vi "TC01 Thermocouple Read.vi"(0 "Physical Channel":tag="Thermocouple1/ai0", 1 "Max Value (deg C)":dbl=100.0, 2 "Min Value (deg C)":dbl, 3 "CJC Source":i32(ring)=10200 items=["Built-In"=10200, "Constant Value"=10116, "Channel"=10113], 4 "CJC Value":dbl=25.0 format="%0.2f", 5 "CJC Channel":refnum<k21>, 6 "Thermocouple Type":i32(ring)=10072 items=["J"=10072, "K"=10073, "N"=10077, "R"=10082, "S"=10085, "T"=10086, "B"=10047, "E"=10055], 7 "Units":i32(ring)=10143 items=["Deg C"=10143, "Deg F"=10144, "Kelvins"=10325, "Deg R"=10145, "From Custom Scale"=10065], 8 "Samples to Average":i32=5 min=1 step=1) -> (20 "Average Read Value":dbl, 21 "Max Read Value":dbl, 22 "Min Read Value":dbl, 23 "Number of reads":i32, 27 "error out":errorcluster)   [LabVIEW 2013]
doc: "This example demonstrates how to continuously acquire temperature measurements using a DAQmx device.\n\nFor instructions on how to connect your signals to the DAQ device, refer to your device documentation."
uses:
  <vilib>/DAQmx/read.llb/DAQmx Read (Analog DBL 1Chan 1Samp).vi
  <vilib>/DAQmx/create/channels.llb/DAQmx Create Channel (AI-Temperature-Thermocouple).vi
  <vilib>/DAQmx/miscellaneous.llb/DAQmx Fill In Error Info.vi
panel:
  out "Approximate\nAcquisition Time":dbl
  out "Waveform Graph":dbl[](graph)
  # "Inputs"
  # "Acquired Data"
  # "Outputs"
  # "Fixed 250mS Sample Rate"
  # "Description of I/O\nInputs:\nMaximum value specifies in units the maximum value you expect to measure. \n \nMinimum value specifies in units the minimum value you expect to measure. \n\nInput Limits (Maximum and Minimum Values)\nInput limits are the maximum and minimum values you expect to measure, after any scaling, including custom scaling. Input limits are sometimes confused with device \nrange. Device range refers only to the input range of a particular device. For instance, the device range for a DAQ device might be 0 to 10 V, but that device might be used \nwith a temperature sensor that outputs 100 mV for every 1 °C. The input limits in that case could be 0 to 100, with 10 V corresponding to 100 °C. \n\nInput limits in a smaller range can improve the precision of your measurement. If, in the previous example, you knew that the temperature would never be higher than \n50 °C, you could choose a minimum value of 0 and a maximum value of 50. The device can then detect smaller differences in temperature because it is digitizing a \nvoltage between 0 and 5 V, rather than 0 and 10 V."
  # "CJC source specifies the source of cold-junction compensation. \n\nChannel (10113) You must use the cjc channel input to specify a channel. \n \nConstant Value (10116) You must use the cjc value input to specify the cold-junction temperature. \n \nInternal (10200) Use a cold-junction compensation channel built into the terminal block. If no such channel is available, this VI returns an error.\n\nCJC value specifies in units the temperature of the cold junction if you set cjc source to Constant Value. \n\nCJC channel specifies the channel that acquires the temperature of the thermocouple cold-junction if you set cjc source to Channel. You can use a global channel or another virtual channel already in the task. If the channel is a temperature channel, NI-DAQmx acquires the temperature in the correct units. Other channel types, such as a resistance channel with a custom sensor, must use a custom scale to scale values to degrees Celsius."
  # "thermocouple type specifies the type of thermocouple connected to the channel. Thermocouple types differ in composition and measurement range. \n\nB (10047) B-type thermocouple. \n \nE (10055) E-type thermocouple. \n \nJ (10072) J-type thermocouple. \n \nK (10073) K-type thermocouple. \n \nN (10077) N-type thermocouple. \n \nR (10082) R-type thermocouple. \n \nS (10085) S-type thermocouple. \n \nT (10086) T-type thermocouple."
  # "units specifies the units to use to return temperature measurements. \n\ndeg C (10143) Degrees Celsius. \n \ndeg F (10144) Degrees Fahrenheit. \n \ndeg R (10145) Degrees Rankine. \n \nFrom Custom Scale (10065) Units a custom scale specifies. If you select this value, you must wire a custom scale name to the custom scale name input. \n \nK (10325) Kelvins."
  # "Samples to Average will capture the specified number of samples to generate an average for the outputs."
  # "Outputs:\nAverage value of samples read\nMax value of samples read\nMin value of samples read\nNumber of samples read\nError cluster"
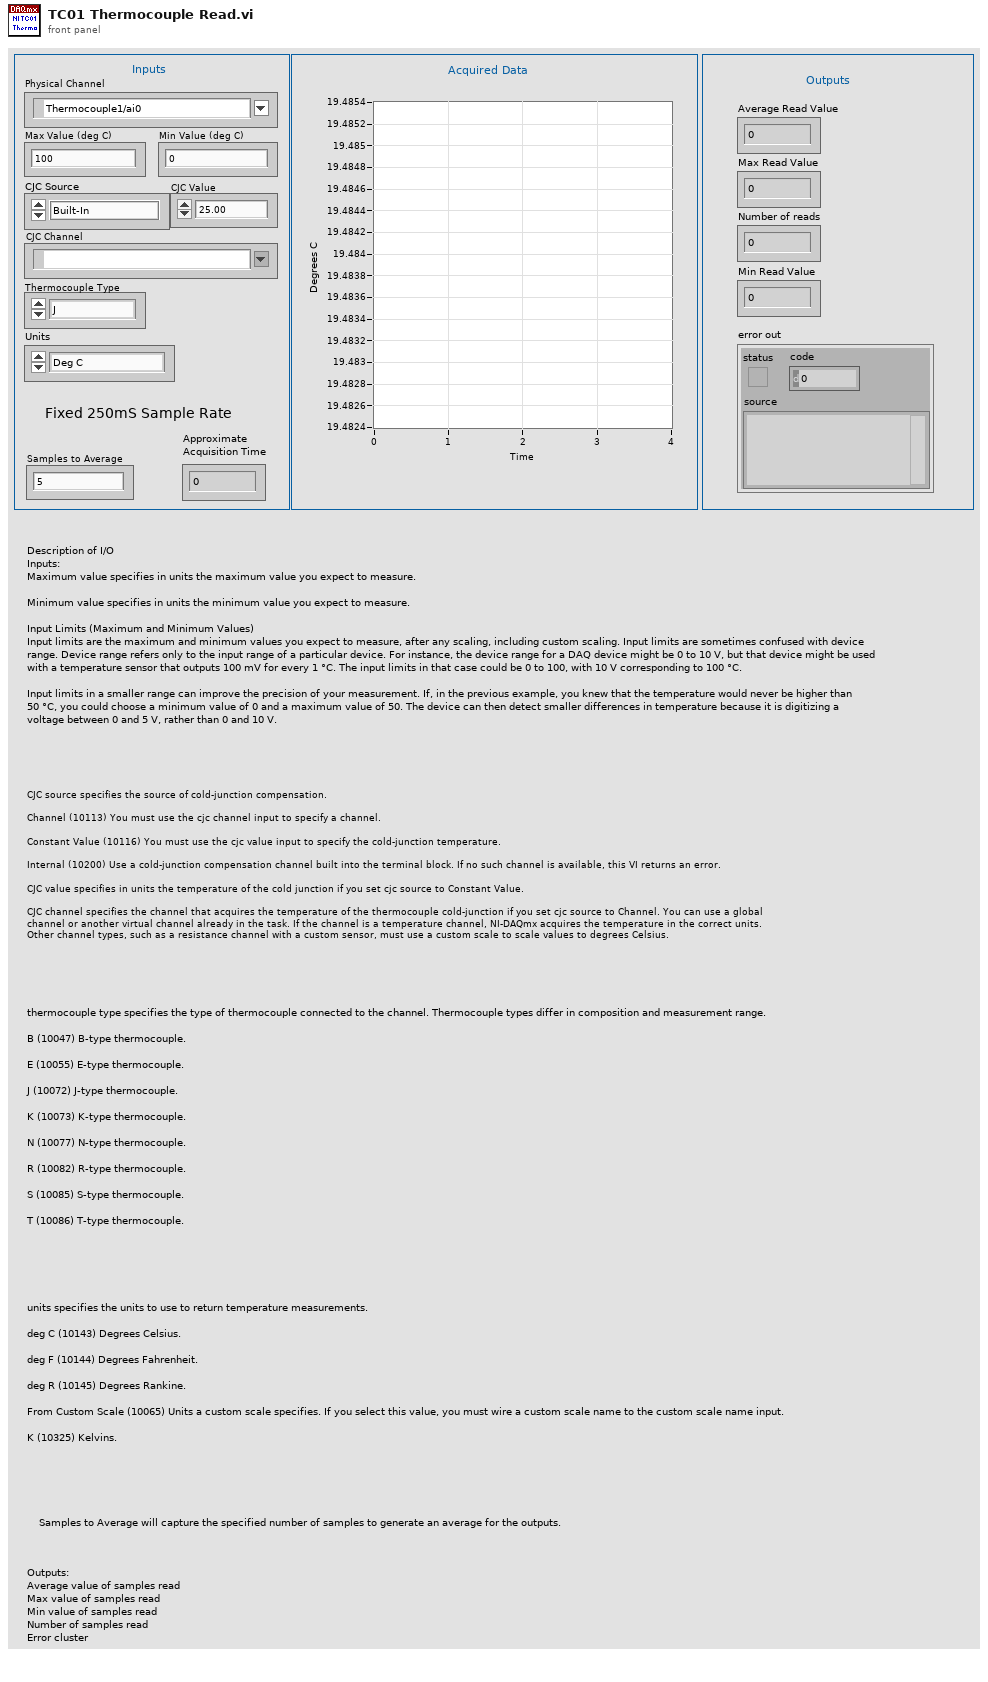
[diagram p1: front panel]
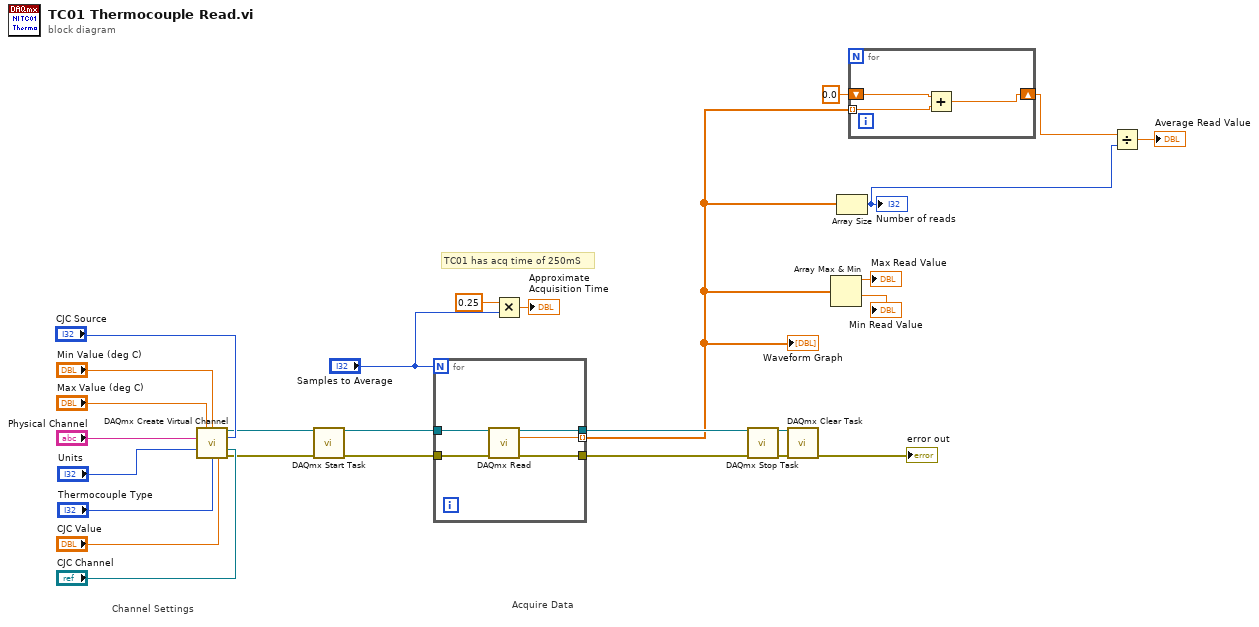
[diagram p0: block diagram]
diagram:
  # "TC01 has acq time of 250mS"
  # "Acquire Data"
  # "Channel Settings"
  n1 = call-poly <vilib>:"DAQmx Create Virtual Channel.vi"("maximum value"="Max Value (deg C)", "minimum value"="Min Value (deg C)", "physical channels"="Physical Channel", "cjc source"="CJC Source", "units"="Units", "cjc channel"="CJC Channel", "thermocouple type"="Thermocouple Type", "cjc value"="CJC Value") -> ("task out"=w6:refnum<k21>, "error out"=w5:errorcluster)  [unwired: 6 in]
  n2 = call <vilib>:"DAQmx Start Task.vi"("task/channels in"=w6, "error in"=w5) -> ("task out"=w27:refnum<k21>, "error out"=w26:errorcluster)  [unwired: 12 in]
  n3 = for {
    N: "Samples to Average" -> [_]
    tunnel: w27 -> [w32]
    tunnel: w26 -> [w31]
    tunnel: [w30] -> w15
    tunnel: [w29] -> w14
    tunnel: [w28] -> w11 mode=indexing
    n4 = call-poly <vilib>:"DAQmx Read.vi"("task/channels in"=w32, "error in"=w31) -> ("task out"=w30:refnum<k21>, "data"=w28:dbl, "error out"=w29:errorcluster)  [unwired: 11 in]
  }
  "Waveform Graph" <- w11
  n5 = Multiply(x=0.25, y="Samples to Average") -> (x*y=→"Approximate\nAcquisition Time":dbl)
  n6 = call <vilib>:"DAQmx Stop Task.vi"("task/channels in"=w15, "error in"=w14) -> ("task out"=w17:refnum<k21>, "error out"=w16:errorcluster)  [unwired: 12 in]
  n7 = call <vilib>:"DAQmx Clear Task.vi"("task in"=w17, "error in"=w16) -> ("error out"=→"error out":errorcluster)  [unwired: 13 in]
  n8 = Array Max & Min(array=w11) -> (max value=→"Max Read Value":dbl, min value=→"Min Read Value":dbl)  [unwired: 2 out]
  n9 = Array Size(array=w11) -> (size(s)=w9:i32)
  "Number of reads" <- w9
  n10 = for {
    shift-right: [w34] -> w10
    shift-left: 0.0 -> [w33]
    tunnel: w11 -> [w35] mode=indexing
    n11 = Add(x=w33, y=w35) -> (x+y=w34:dbl)
  }
  n12 = Divide(x=w10, y=w9) -> (x/y=→"Average Read Value":dbl)
